vi "measure Permit Range.vi"(8 "error in (no error)":errorcluster, 11 "SA Measurement in":refnum<class "SA Measurement.lvclass">) -> (0 "error out":errorcluster, 3 "SA Measurement out":refnum<class "SA Measurement.lvclass">)   [LabVIEW 2023, in "Spectrum Analyzer.lvlib" / "SA Measurement.lvclass"]
uses:
  SA Measurement.lvclass
  SA Measurement.lvclass/SA Measurement.ctl
  TYPE DEFINITION/Keysight 9020A/TYPE Measurement Preset.ctl
  Spectrum Analyzer.lvlib
  TYPE DEFINITION/TYPE RBW and VBW Select.ctl
  Interface_Spectrum/Interface_Spectrum.lvclass
  TYPE DEFINITION/TYPE Marker Peak Search Type.ctl
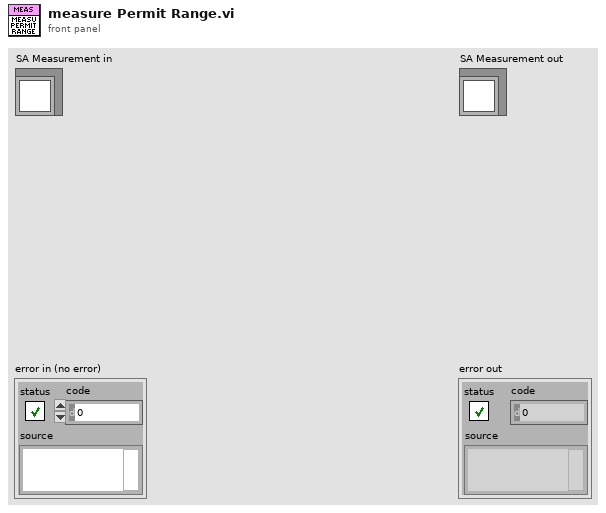
[diagram p1: front panel]
types:
  T1 = typedef "Spectrum Analyzer.lvlib/TYPE Marker Peak Search Type.ctl" = enum16{"Max", "Next Peak"}
  T2 = enum16{"Free Run", "Video (IF Envelop)", "RF Burst"}
  T3 = typedef "Spectrum Analyzer.lvlib/TYPE RBW and VBW Select.ctl" = enum16{"Res BW", "Video BW"}
  T4 = typedef "Spectrum Analyzer.lvlib/TYPE Measurement Preset.ctl" = enum16{"Sweep SA Mode", "Channel Power", "Occupied BW", "ACP", "Spurious Emission", "Spurious Emission Mask", "Burst Power (Transmit Power)"}
  T5 = typedef "Spectrum Analyzer.lvlib/TYPE Y-axis Unit.ctl" = enum16{"dBm", "dBmV", "dBuV", "dBpW", "Volt", "Ampere", "Watt"}
  T6 = typedef "Spectrum Analyzer.lvlib/TYPE Reference Level and Atten Param.ctl" = cluster{"Reference Level":dbl, "Atten":i32, "Atten Auto?":bool, "Reference Level Offset":dbl}
  T7 = typedef "Spectrum Analyzer.lvlib/TYPE Display Trace Mode Select.ctl" = enum16{"Clear Write", "Max Hold", "Min Hold", "Average", "View"}
  T8 = typedef "Spectrum Analyzer.lvlib/TYPE Detect Mode Select.ctl" = enum16{"Det Auto (Normal)", "Auto Peak", "Positive Peak", "Negative Peak", "Sample", "RMS", "Average", "Quasipeak", "CISPR Average", "RMS Average"}
  T9 = cluster{"Trace Mode":T7, "Detector Type":T8, "Detect Auto?":bool}[]
  T10 = typedef "Spectrum Analyzer.lvlib/TYPE Average Mode Select.ctl" = enum16{"Linear(Voltage Avg)", "Video(Log)", "Power"}
  T11 = typedef "Spectrum Analyzer.lvlib/TYPE Marker Value.ctl" = cluster{"X-axis":dbl, "Y-axis":dbl}
  T12 = typedef "Spectrum Analyzer.lvlib/TYPE Trace Value Array.ctl" = cluster{"Frequency":dbl[], "Amplitude":dbl[]}
  T13 = cluster{"Permit Range Frequency (Hz)":dbl, "Valid?":bool}
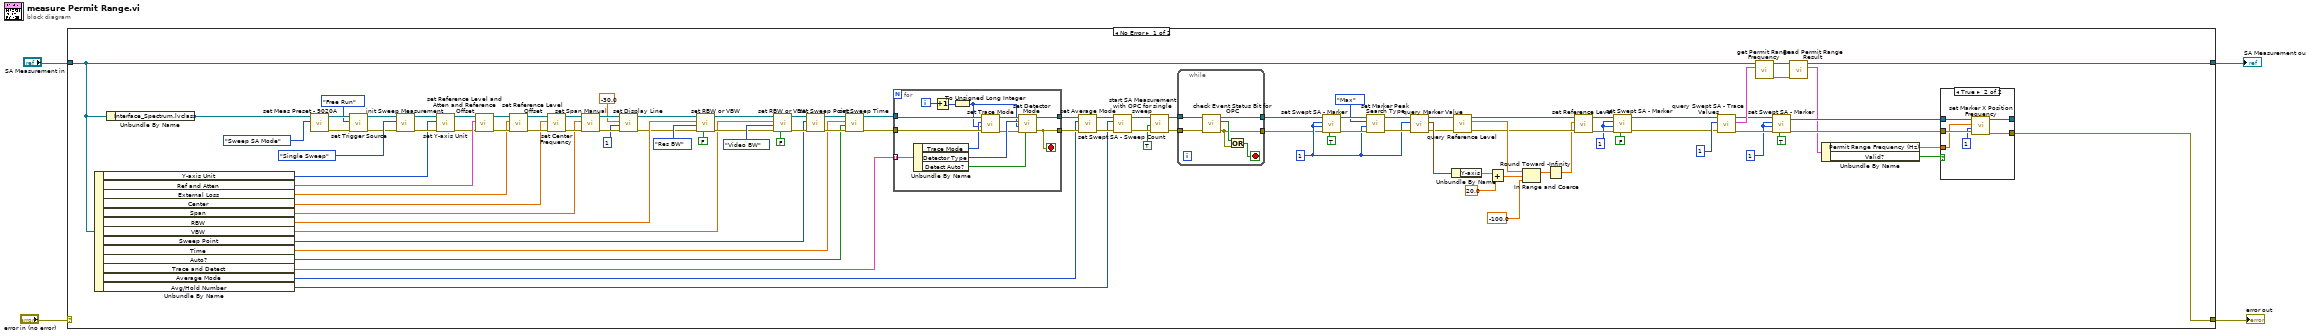
[diagram p0: block diagram]
diagram:
  n1 = case shown="No Error" "error in (no error)" {
    selector: "error in (no error)" -> [_ w134]
    tunnel: [w32 w134] -> w1
    tunnel: [w33 w133] -> w3
    tunnel: "SA Measurement in" -> [w45 w133]
    frame No Error {
      w9 = 1 ("Index")
      w25 = 1 ("Index")
      w39 = 1 ("Index")
      n2 = Unbundle By Name(w45) -> ("Y-axis Unit"=w80:T5, "Ref and Atten"=w102:T6, "External Loss"=w99:dbl, "Center"=w96:dbl, "Span"=w93:dbl, "RBW"=w92:dbl, "VBW"=w85:dbl, "Sweep Point"=w77:u32, "Time"=w74:dbl, "Auto?"=w73:bool, "Trace and Detect"=w70:T9, "Average Mode"=w67:T10, "Avg/Hold Number"=w64:u32)
      n3 = Unbundle By Name(w45) -> ("Interface_Spectrum.lvclass"=w105:refnum<class "Interface_Spectrum.lvclass">)
      n4 = call-dynamic "set Meas Preset - 9020A.vi"("Measurement Preset"=TYPE_Measurement_Preset."Sweep SA Mode", "Interface_Spectrum in"=w105) -> ("error out"=w56:errorcluster, "Interface_Spectrum out"=w57:refnum<class "Interface_Spectrum.lvclass">)  [unwired: 8 in]
      n5 = call-dynamic "set Trigger Source.vi"("error in (no error)"=w56, "Trigger Source"=T2."Free Run", "Interface_Spectrum in"=w57) -> ("error out"=w53:errorcluster, "Interface_Spectrum out"=w54:refnum<class "Interface_Spectrum.lvclass">)  [unwired: 7 in]
      n6 = call-dynamic "init Sweep Measurement.vi"("error in (no error)"=w53, "Sweep Measurement Mode"=enum16{"Single Sweep", "Continuous Sweep"}."Single Sweep", "Interface_Spectrum in"=w54) -> ("error out"=w83:errorcluster, "Interface_Spectrum out"=w84:refnum<class "Interface_Spectrum.lvclass">)  [unwired: 7 in]
      n7 = call-dynamic "set Y-axis Unit.vi"("error in (no error)"=w83, "Y-axis Unit"=w80, "Interface_Spectrum in"=w84) -> ("error out"=w81:errorcluster, "Interface_Spectrum out"=w82:refnum<class "Interface_Spectrum.lvclass">)  [unwired: 7 in]
      n8 = call-dynamic "set Reference Level and Atten and Reference Offset.vi"("error in (no error)"=w81, "Reference Level, Atten, Reference Offset"=w102, "Interface_Spectrum in"=w82) -> ("error out"=w100:errorcluster, "Interface_Spectrum out"=w101:refnum<class "Interface_Spectrum.lvclass">)  [unwired: 7 in]
      n9 = call-dynamic "set Reference Level Offset.vi"("error in (no error)"=w100, "Reference Level Offset"=w99, "Interface_Spectrum in"=w101) -> ("error out"=w97:errorcluster, "Interface_Spectrum out"=w98:refnum<class "Interface_Spectrum.lvclass">)  [unwired: 7 in]
      n10 = call-dynamic "set Center Frequency.vi"("error in (no error)"=w97, "Center Frequency (Hz)"=w96, "Interface_Spectrum in"=w98) -> ("error out"=w94:errorcluster, "Interface_Spectrum out"=w95:refnum<class "Interface_Spectrum.lvclass">)  [unwired: 7 in]
      n11 = call-dynamic "set Span Manual.vi"("error in (no error)"=w94, "Span (Hz)"=w93, "Interface_Spectrum in"=w95) -> ("error out"=w51:errorcluster, "Interface_Spectrum out"=w52:refnum<class "Interface_Spectrum.lvclass">)  [unwired: 7 in]
      n12 = call-dynamic "set Display Line.vi"("error in (no error)"=w51, "Line Index"=1, "Amplitude"=-30.0, "Interface_Spectrum in"=w52) -> ("error out"=w47:errorcluster, "Interface_Spectrum out"=w48:refnum<class "Interface_Spectrum.lvclass">)  [unwired: 6 in]
      n13 = call-dynamic "set RBW or VBW.vi"("BW Auto?"=FALSE, "error in (no error)"=w47, "BW Type"=TYPE_RBW_and_VBW_Select."Res BW", "BW Value (Hz)"=w92, "Interface_Spectrum in"=w48) -> ("error out"=w86:errorcluster, "Interface_Spectrum out"=w87:refnum<class "Interface_Spectrum.lvclass">)  [unwired: 5 in]
      n14 = call-dynamic "set RBW or VBW.vi"("BW Auto?"=FALSE, "error in (no error)"=w86, "BW Type"=TYPE_RBW_and_VBW_Select."Video BW", "BW Value (Hz)"=w85, "Interface_Spectrum in"=w87) -> ("error out"=w78:errorcluster, "Interface_Spectrum out"=w79:refnum<class "Interface_Spectrum.lvclass">)  [unwired: 5 in]
      n15 = call-dynamic "set Sweep Point.vi"("error in (no error)"=w78, "Sweep Point"=w77, "Interface_Spectrum in"=w79) -> ("error out"=w75:errorcluster, "Interface_Spectrum out"=w76:refnum<class "Interface_Spectrum.lvclass">)  [unwired: 7 in]
      n16 = call-dynamic "set Sweep Time.vi"("error in (no error)"=w75, "Sweep Time Auto?"=w73, "Sweep Time(sec)"=w74, "Interface_Spectrum in"=w76) -> ("error out"=w71:errorcluster, "Interface_Spectrum out"=w72:refnum<class "Interface_Spectrum.lvclass">)  [unwired: 6 in]
      n17 = for {
        tunnel: w72 -> [w131]
        tunnel: w71 -> [w130]
        tunnel: w70 -> [w132] mode=indexing
        tunnel: [w120] -> w68
        tunnel: [w121] -> w69
        i -> [w129]
        stop <- w120 stop-if-true
        n18 = Unbundle By Name(w132) -> ("Trace Mode"=w127:T7, "Detector Type"=w125:T8, "Detect Auto?"=w122:bool)
        n19 = Increment(x=w129) -> (x+1=w128:i32)
        n20 = To Unsigned Long Integer(number=w128) -> (unsigned 32bit integer=w123:u32)
        n21 = call-dynamic "set Trace Mode.vi"("error in (no error)"=w130, "Trace Index"=w123, "Trace Mode"=w127, "Interface_Spectrum in"=w131) -> ("error out"=w124:errorcluster, "Interface_Spectrum out"=w126:refnum<class "Interface_Spectrum.lvclass">)  [unwired: 6 in]
        n22 = call-dynamic "set Detector Mode.vi"("Detect Auto?"=w122, "error in (no error)"=w124, "Trace Index"=w123, "Detector Type"=w125, "Interface_Spectrum in"=w126) -> ("error out"=w120:errorcluster, "Interface_Spectrum out"=w121:refnum<class "Interface_Spectrum.lvclass">)  [unwired: 5 in]
      }
      n23 = call-dynamic "set Average Mode.vi"("error in (no error)"=w68, "Average Mode"=w67, "Interface_Spectrum in"=w69) -> ("error out"=w65:errorcluster, "Interface_Spectrum out"=w66:refnum<class "Interface_Spectrum.lvclass">)  [unwired: 7 in]
      n24 = call-dynamic "set Swept SA - Sweep Count.vi"("error in (no error)"=w65, "Sweep Count"=w64, "Interface_Spectrum in"=w66) -> ("error out"=w62:errorcluster, "Interface_Spectrum out"=w63:refnum<class "Interface_Spectrum.lvclass">)  [unwired: 7 in]
      n25 = call-dynamic "start SA Measurement with OPC for single sweep.vi"("error in (no error)"=w62, "with OPC?"=TRUE, "Interface_Spectrum in"=w63) -> ("error out"=w59:errorcluster, "Interface_Spectrum out"=w60:refnum<class "Interface_Spectrum.lvclass">)  [unwired: 7 in]
      n26 = while {
        tunnel: w60 -> [w119]
        tunnel: w59 -> [w118]
        tunnel: [w115] -> w7
        tunnel: [w114] -> w8
        stop <- w116 stop-if-true
        n27 = call-dynamic "check Event Status Bit for OPC.vi"("error in (no error)"=w118, "Interface_Spectrum in"=w119) -> ("error out"=w115:errorcluster, "OPC Bit Changed?"=w117:bool, "Interface_Spectrum out"=w114:refnum<class "Interface_Spectrum.lvclass">)  [unwired: 7 in]
        n28 = Or(x=w117, y=w115) -> (x .or. y?=w116:bool)
      }
      n29 = call-dynamic "set Swept SA - Marker.vi"("On?"=TRUE, "error in (no error)"=w7, "trace"=w25, "Index"=w25, "Interface_Spectrum in"=w8) -> ("error out"=w29:errorcluster, "Interface_Spectrum out"=w30:refnum<class "Interface_Spectrum.lvclass">)  [unwired: 5 in]
      n30 = call-dynamic "set Marker Peak Search Type.vi"("error in (no error)"=w29, "Marker Index"=w25, "Peak Search Type"=TYPE_Marker_Peak_Search_Type."Max", "Interface_Spectrum in"=w30) -> ("error out"=w26:errorcluster, "Interface_Spectrum out"=w27:refnum<class "Interface_Spectrum.lvclass">)  [unwired: 6 in]
      n31 = call-dynamic "query Marker Value.vi"("error in (no error)"=w26, "Marker Index"=w25, "Interface_Spectrum in"=w27) -> ("error out"=w20:errorcluster, "Marker Value"=w22:T11, "Interface_Spectrum out"=w21:refnum<class "Interface_Spectrum.lvclass">)  [unwired: 6 in]
      n32 = Unbundle By Name(w22) -> ("Y-axis"=w24:dbl)
      n33 = call-dynamic "query Reference Level.vi"("error in (no error)"=w20, "Interface_Spectrum in"=w21) -> ("error out"=w15:errorcluster, "Ref Level"=w18:dbl, "Interface_Spectrum out"=w19:refnum<class "Interface_Spectrum.lvclass">)  [unwired: 7 in]
      n34 = Add(x=w24, y=20.0) -> (x+y=w17:dbl)
      n35 = In Range and Coerce(upper limit=w18, x=w17, lower limit=-100.0) -> (coerced(x)=w14:dbl)  [unwired: 1 out]
      n36 = Round Toward -Infinity(1:w14) -> (0:w13:dbl)
      n37 = call-dynamic "set Reference Level.vi"("error in (no error)"=w15, "Reference Level"=w13, "Interface_Spectrum in"=w19) -> ("error out"=w11:errorcluster, "Interface_Spectrum out"=w12:refnum<class "Interface_Spectrum.lvclass">)  [unwired: 7 in]
      n38 = call-dynamic "set Swept SA - Marker.vi"("On?"=FALSE, "error in (no error)"=w11, "trace"=w9, "Index"=w9, "Interface_Spectrum in"=w12) -> ("error out"=w5:errorcluster, "Interface_Spectrum out"=w6:refnum<class "Interface_Spectrum.lvclass">)  [unwired: 5 in]
      n39 = call-dynamic "query Swept SA - Trace Values.vi"("error in (no error)"=w5, "Trace Index"=u32 1, "Interface_Spectrum in"=w6) -> ("error out"=w42:errorcluster, "Trace Values"=w44:T12, "Interface_Spectrum out"=w43:refnum<class "Interface_Spectrum.lvclass">)  [unwired: 6 in]
      n40 = call "get Permit Range Frequency.vi"("Trace Values"=w44, "SA Measurement in"=w45) -> ("error out"=w37:errorcluster, "SA Measurement out"=w38:refnum<class "SA Measurement.lvclass">)  [unwired: 8 in]
      n41 = call-dynamic "set Swept SA - Marker.vi"("On?"=TRUE, "error in (no error)"=w42, "trace"=w39, "Index"=w39, "Interface_Spectrum in"=w43) -> ("error out"=w40:errorcluster, "Interface_Spectrum out"=w41:refnum<class "Interface_Spectrum.lvclass">)  [unwired: 5 in]
      n42 = call "Read Permit Range Result.vi"("error in (no error)"=w37, "SA Measurement in"=w38) -> ("Permit Range Result"=w36:T13, "SA Measurement out"=w33:refnum<class "SA Measurement.lvclass">)  [unwired: 7 in, 1 out]
      n43 = Unbundle By Name(w36) -> ("Permit Range Frequency (Hz)"=w34:dbl, "Valid?"=w35:bool)
      n44 = case shown="True" w35 {
        tunnel: w41 -> [w107 w113]
        tunnel: w40 -> [w106 w112]
        tunnel: w34 -> [_ w111]
        tunnel: [w107 w109] -> _
        tunnel: [w106 w108] -> w32
        frame False {
        }
        frame True {
          n45 = call-dynamic "set Marker X Position Frequency.vi"("error in (no error)"=w112, "Index"=1, "X Position Frequency (Hz)"=w111, "Interface_Spectrum in"=w113) -> ("error out"=w108:errorcluster, "Interface_Spectrum out"=w109:refnum<class "Interface_Spectrum.lvclass">)  [unwired: 6 in]
        }
      }
    }
    frame Error {
    }
  }
  "error out" <- w1
  "SA Measurement out" <- w3
